vi "Initialise.vi"(8 "error in (no error)":errorcluster, 11 "ChangeNotifier in":refnum<class "ChangeNotifier.lvclass">) -> (0 "error out":errorcluster, 3 "ChangeNotifier out":refnum<class "ChangeNotifier.lvclass">)   [LabVIEW 2024, in "ChangeNotifier.lvclass"]
doc: "Initialise ChangeNotifier with notifyChanges event which can be registered so reactive updates can be made."
uses:
  ChangeNotifier.lvclass
  ChangeNotifier.lvclass/ChangeNotifier.ctl
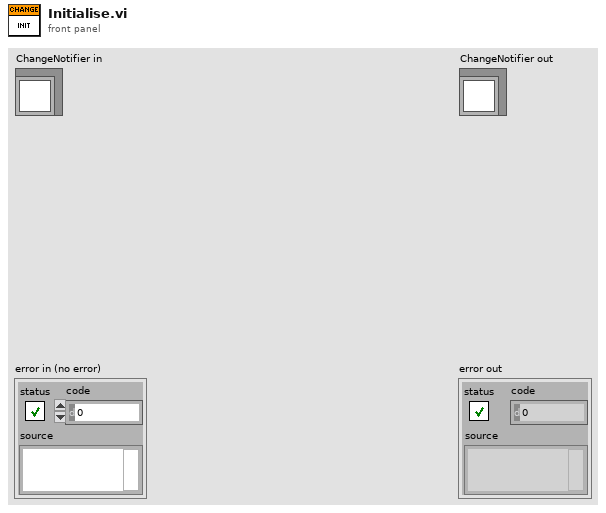
[diagram p1: front panel]
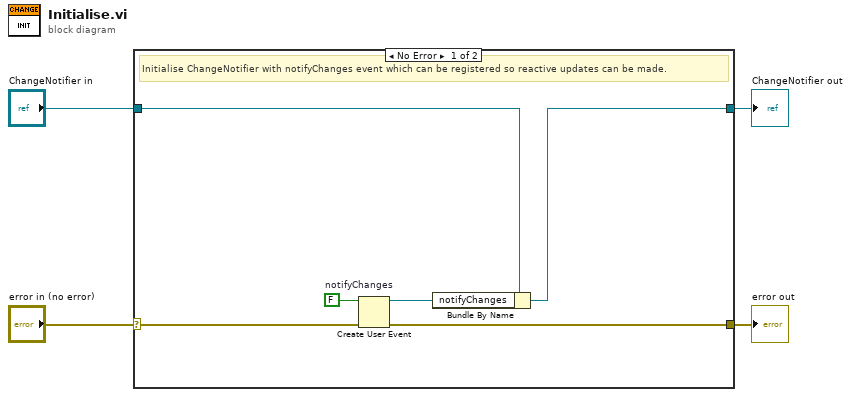
[diagram p0: block diagram]
diagram:
  n1 = case shown="No Error" "error in (no error)" {
    selector: "error in (no error)" -> [w7 w12]
    tunnel: [w6 w12] -> w3
    tunnel: [w5 w11] -> w1
    tunnel: "ChangeNotifier in" -> [w8 w11]
    frame No Error {
      w10 = FALSE  # notifyChanges
      # "Initialise ChangeNotifier with notifyChanges event which can be registered so reactive updates can be made."
      n2 = Create User Event(user event datatype=w10, error in=w7) -> (user event=w9:refnum<user-event>, error out=w6:errorcluster)
      n3 = Bundle By Name(cluster=w8, "notifyChanges"=w9) -> (w5:refnum<class "ChangeNotifier.lvclass">)
    }
    frame Error {
    }
  }
  "error out" <- w3
  "ChangeNotifier out" <- w1
